vi "FuncVI_Sub - Script - Get Script File Content.vi"(7 "Caller CSE RefNum":T1, 10 "Check Script TS (T)":bool=TRUE, 11 "Script name":string) -> (0 "error out":errorcluster, 2 "Script body":string, 3 "Script Path":path)   [LabVIEW 2021]
doc: "::: CalcExpress Toolkit :::\nCopyright (c) 2000-2026 Konstantin Shifershteyn. All rights reserved."
uses:
  cse.llb/CSE Instance RefNum.ctl
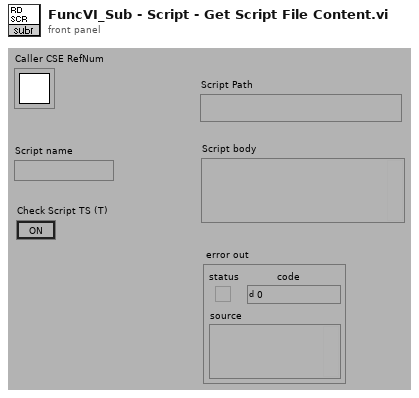
[diagram p1: front panel]
types:
  T1 = typedef "CSE Instance RefNum.ctl" = refnum<k1>
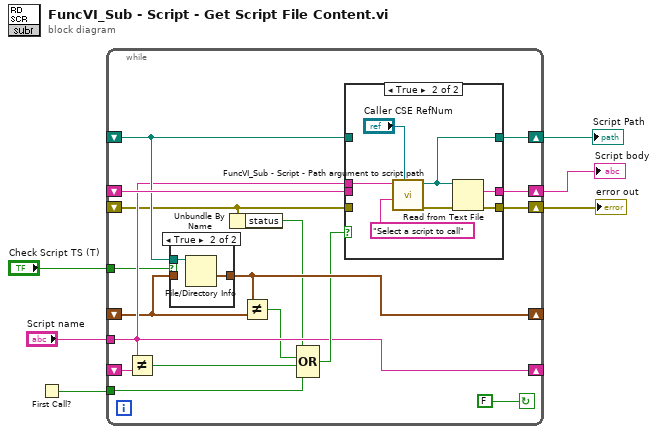
[diagram p0: block diagram]
diagram:
  n1 = First Call?() -> (First Call?: T/F=w2:bool)
  n2 = while {
    shift-right: [w23] -> w5
    shift-left: _ -> [w19]
    shift-right: [w20] -> w4
    shift-left: _ -> [w18]
    shift-right: [w22] -> w6
    shift-left: _ -> [w10]
    tunnel: "Script name" -> [w14]
    shift-right: [w17] -> _
    shift-left: _ -> [w8]
    shift-right: [w14] -> _
    shift-left: _ -> [w15]
    tunnel: w2 -> [w11]
    tunnel: "Check Script TS (T)" -> [w7]
    stop <- FALSE continue-if-true
    n3 = Not Equal?(x=w14, y=w15) -> (x != y?=w13:bool)
    n4 = case shown="True" w7 {
      tunnel: w18 -> [_ w26]
      tunnel: [w24 w25] -> w17
      tunnel: w8 -> [w24 _]
      frame False {
      }
      frame True {
        n5 = File/Directory Info(path=w26) -> (last mod=w25:timestamp)  [unwired: 1 in, 6 out]
      }
    }
    n6 = Unbundle By Name(w10) -> ("status"=w9:bool)
    n7 = Not Equal?(x=w17, y=w8) -> (x != y?=w12:bool)
    n8 = Compound Arithmetic op=OR(w9, w12, w13, w11) -> (w16:bool)
    n9 = case shown="True" w16 {
      tunnel: [w29 w36] -> w23
      tunnel: w10 -> [w27 _]
      tunnel: [w27 w35] -> w22
      tunnel: [w28 w34] -> w20
      tunnel: w19 -> [w29 _]
      tunnel: w18 -> [w28 _]
      tunnel: w14 -> [_ w32]
      frame False {
      }
      frame True {
        n10 = call "FuncVI_Sub - Script - Path argument to script path.vi"("CSE RefNum"="Caller CSE RefNum", "prompt"="Select a script to call", "arg: path"=w32) -> ("error out"=w33:errorcluster, "script path"=w34:path)  [unwired: 7 in]
        n11 = Read from Text File(file (use dialog)=w34, error in=w33) -> (text=w36:string, error out=w35:errorcluster)  [unwired: 2 in, 2 out]
      }
    }
  }
  "Script Path" <- w4
  "Script body" <- w5
  "error out" <- w6
